vi "FX_ReadWords.vi"(8 "error in (no error)":errorcluster, 9 "Count":u16, 10 "Device":string, 11 "PLC Conn":refnum<visa-resource-name>) -> (1 "error out":errorcluster, 2 "Words":u16[](array[numeric]), 3 "PLC Conn out":refnum<visa-resource-name>)   [LabVIEW 2026]
doc: "Use this template to build a VI to use as a subVI."
panel:
  # "ÕfÃ÷£º×x D¡£D0 Î»Ö· 1000h£¬Ã¿‚€ D ƒÉÎ»Ôª½M£¬µÍÎ»Ôª½MÔÚ\nÇ°¡£Ã¿´Î×î¶à 64 Î»Ôª½M¡£"
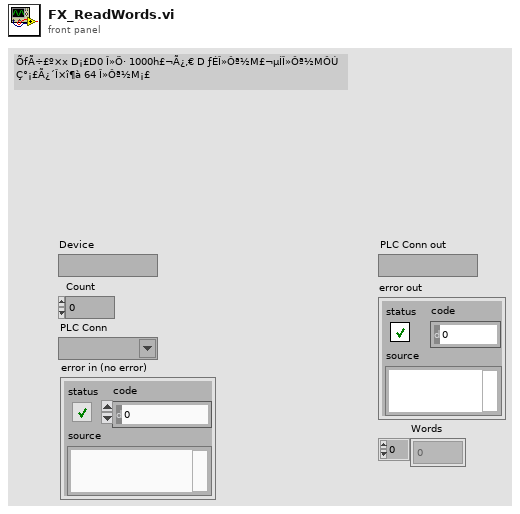
[diagram p1: front panel]
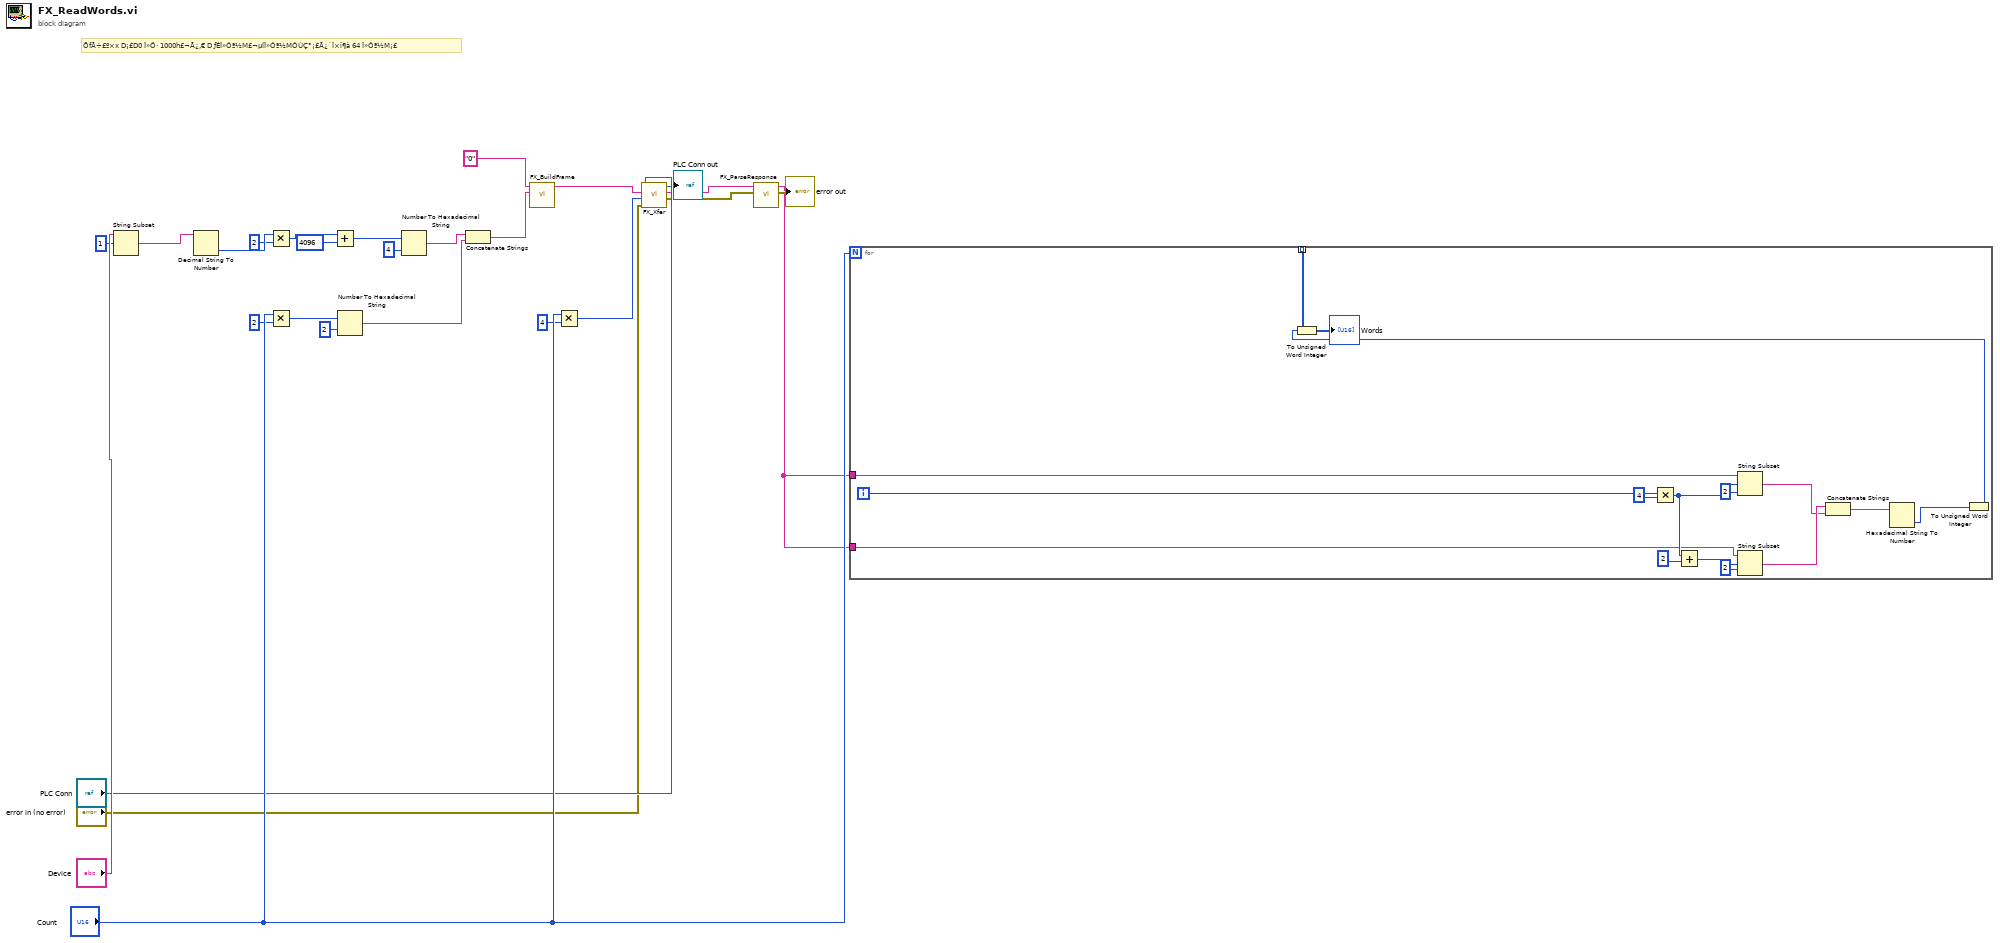
[diagram p0: block diagram]
diagram:
  # "ÕfÃ÷£º×x D¡£D0 Î»Ö· 1000h£¬Ã¿‚€ D ƒÉÎ»Ôª½M£¬µÍÎ»Ôª½MÔÚÇ°¡£Ã¿´Î×î¶à 64 Î»Ôª½M¡£"
  n1 = String Subset(string="Device", offset (0)=1) -> (substring=w26:string)  [unwired: 1 in]
  n2 = Decimal String To Number(string=w26) -> (number=w25:i32)  [unwired: 2 in, 1 out]
  n3 = Multiply(x=w25, y=2) -> (x*y=w23:i32)
  n4 = Multiply(x="Count", y=u16 2) -> (x*y=w17:u16)
  n5 = Add(x=w23, y=4096) -> (x+y=w21:i32)
  n6 = Number To Hexadecimal String(1:i16 2 ("width (-)"), 2:w17) -> (0:w14:string)
  n7 = Number To Hexadecimal String(1:i16 4 ("width (-)"), 2:w21) -> (0:w15:string)
  n8 = Concatenate Strings(w15, w14) -> (w13:string)
  n9 = call "FX_BuildFrame.vi"("Content"=w13, "Command"="0") -> ("Frame"=w12:string)  [unwired: 9 in]
  n10 = Multiply(x="Count", y=u16 4) -> (x*y=w8:u16)
  n11 = call "FX_Xfer.vi"("error in (no error)"="error in (no error)", "Data Chars"=w8, "TX"=w12, "PLC Conn"="PLC Conn") -> ("error out"=w6:errorcluster, "RX"=w7:string, "PLC Conn out"=→"PLC Conn out":refnum<visa-resource-name>)  [unwired: 5 in]
  n12 = call "FX_ParseResponse.vi"("error in (no error)"=w6, "RX"=w7) -> ("error out"=→"error out":errorcluster, "Data"=w3:string)  [unwired: 8 in]
  n13 = for {
    N: "Count" -> [_]
    tunnel: w3 -> [w41]
    tunnel: w3 -> [w37]
    tunnel: [w30] -> w2 mode=indexing
    i -> [w43]
    n14 = Multiply(x=w43, y=4) -> (x*y=w40:i32)
    n15 = Add(x=w40, y=2) -> (x+y=w36:i32)
    n16 = String Subset(string=w41, offset (0)=w40, length (rest)=2 ("length (rest)")) -> (substring=w33:string)
    n17 = String Subset(string=w37, offset (0)=w36, length (rest)=2 ("length (rest)")) -> (substring=w34:string)
    n18 = Concatenate Strings(w34, w33) -> (w32:string)
    n19 = Hexadecimal String To Number(string=w32) -> (number=w31:u32)  [unwired: 2 in, 1 out]
    n20 = To Unsigned Word Integer(number=w31) -> (unsigned 16bit integer=w30:u16)
  }
  n21 = To Unsigned Word Integer(number=w2) -> (unsigned 16bit integer=→"Words":u16[])
